vi "Lockin.Low Pass Filter Bank.vi"(6 "Butterworth? [T]":bool=TRUE, 8 "error in (no error)":errorcluster, 10 "WFms in":waveform(dbl)[](array[waveform]), 11 "DSP in":refnum<class "DSP.lvclass">) -> (0 "error out":errorcluster, 2 "Wfms out":waveform(dbl)[](array[waveform]))   [LabVIEW 2019, in "DSP.lvclass"]
uses:
  DSP.lvclass
  DSP.lvclass/DSP.ctl
  Create Low Pass RC Filter (FGV).vi
  Create Low Pass Filter (FGV).vi
  DFD Filter Array.vi
  Waveform.Attributes/Waveform.Attributes.lvlib
panel:
  out "DSP out":refnum<class "DSP.lvclass">
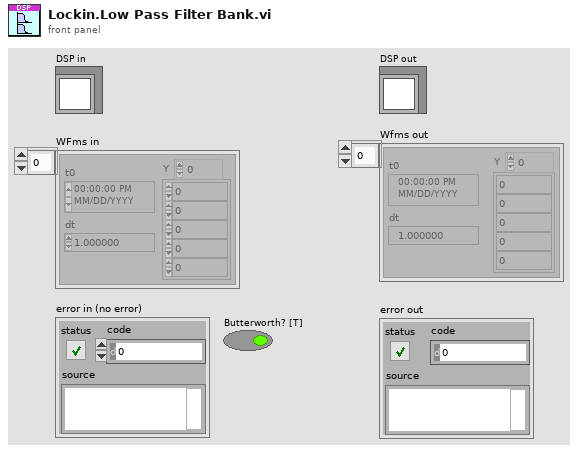
[diagram p1: front panel]
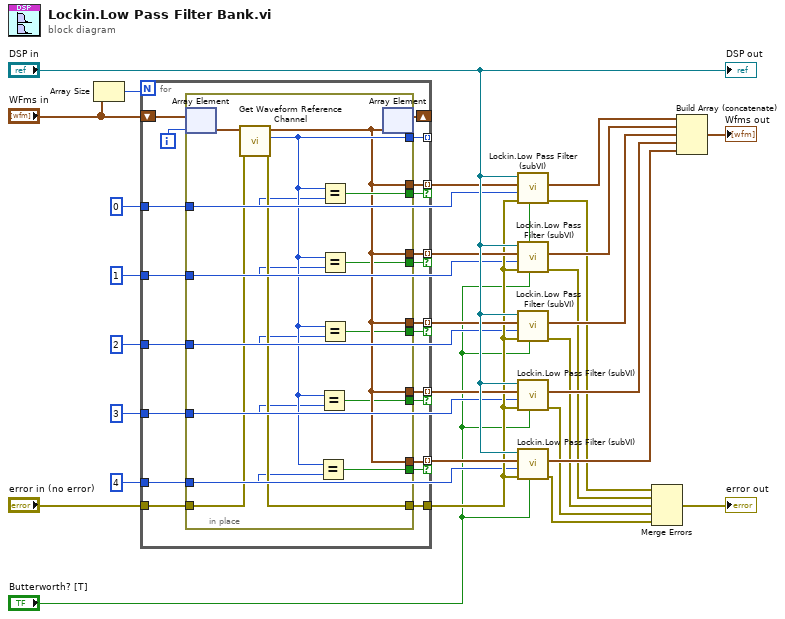
[diagram p0: block diagram]
diagram:
  w6 = 4 ("y")
  w5 = 3 ("y")
  w4 = 2 ("y")
  w3 = 1 ("y")
  w2 = 0 ("y")
  n1 = Array Size(array="WFms in") -> (size(s)=w26:i32)
  n2 = for {
    N: w26 -> [_]
    shift-right: [w44] -> _
    shift-left: "WFms in" -> [w48]
    tunnel: [w45] -> _ mode=indexing
    tunnel: "error in (no error)" -> [w47]
    tunnel: [w46] -> w7
    tunnel: [w43] -> w12 mode=indexing if=w42
    tunnel: [w41] -> w11 mode=indexing if=w34
    tunnel: [w40] -> w10 mode=indexing if=w35
    tunnel: [w39] -> w9 mode=indexing if=w36
    tunnel: [w38] -> w8 mode=indexing if=w37
    tunnel: w6 -> [w33]
    tunnel: w5 -> [w32]
    tunnel: w4 -> [w31]
    tunnel: w3 -> [w30]
    tunnel: w2 -> [w29]
    i -> [w49]
    n3 = in-place {
      in-place-border: w47 -> [w63]
      in-place-border: [w62] -> w46
      in-place-border: [w61] -> w45
      in-place-border: [w59] -> w43
      in-place-border: [w60] -> w42
      in-place-border: [w59] -> w41
      in-place-border: [w59] -> w40
      in-place-border: [w59] -> w39
      in-place-border: [w59] -> w38
      in-place-border: [w58] -> w37
      in-place-border: [w57] -> w36
      in-place-border: [w56] -> w35
      in-place-border: [w55] -> w34
      in-place-border: w33 -> [w54]
      in-place-border: w32 -> [w53]
      in-place-border: w31 -> [w52]
      in-place-border: w30 -> [w51]
      in-place-border: w29 -> [w50]
      n4 = in-place-array #1(w48, w49) -> (w64:waveform(dbl))
      n5 = call "Get Waveform Reference Channel.vi"("error in (no error)"=w63, "Reference in"=w64) -> ("error out"=w62:errorcluster, "Reference Channel"=w61:i32, "Reference out"=w59:waveform(dbl))  [unwired: 7 in]
      n6 = Equal?(x=w61, y=w54) -> (x = y?=w58:bool)
      n7 = Equal?(x=w61, y=w53) -> (x = y?=w57:bool)
      n8 = Equal?(x=w61, y=w50) -> (x = y?=w60:bool)
      n9 = Equal?(x=w61, y=w51) -> (x = y?=w55:bool)
      n10 = Equal?(x=w61, y=w52) -> (x = y?=w56:bool)
      n11 = in-place-array #1(w59) -> (w44:waveform(dbl)[])  [unwired: 1 out]
    }
  }
  n12 = call "Lockin.Low Pass Filter (subVI).vi"("Butterworth? [T]"="Butterworth? [T]", "error in (no error)"=w7, "Element Data"=w2, "signal in"=w12, "DSP in"="DSP in") -> ("error out"=w14:errorcluster, "signal out"=w13:waveform(dbl)[])  [unwired: 3 in, 2 out]
  n13 = call "Lockin.Low Pass Filter (subVI).vi"("Butterworth? [T]"="Butterworth? [T]", "error in (no error)"=w7, "Element Data"=w3, "signal in"=w11, "DSP in"="DSP in") -> ("error out"=w18:errorcluster, "signal out"=w19:waveform(dbl)[])  [unwired: 3 in, 2 out]
  n14 = call "Lockin.Low Pass Filter (subVI).vi"("Butterworth? [T]"="Butterworth? [T]", "error in (no error)"=w7, "Element Data"=w4, "signal in"=w10, "DSP in"="DSP in") -> ("error out"=w17:errorcluster, "signal out"=w20:waveform(dbl)[])  [unwired: 3 in, 2 out]
  n15 = call "Lockin.Low Pass Filter (subVI).vi"("Butterworth? [T]"="Butterworth? [T]", "error in (no error)"=w7, "Element Data"=w5, "signal in"=w9, "DSP in"="DSP in") -> ("error out"=w16:errorcluster, "signal out"=w21:waveform(dbl)[])  [unwired: 3 in, 2 out]
  n16 = call "Lockin.Low Pass Filter (subVI).vi"("Butterworth? [T]"="Butterworth? [T]", "error in (no error)"=w7, "Element Data"=w6, "signal in"=w8, "DSP in"="DSP in") -> ("error out"=w15:errorcluster, "signal out"=w22:waveform(dbl)[])  [unwired: 3 in, 2 out]
  n17 = Merge Errors(w14, w18, w17, w16, w15) -> (→"error out":errorcluster)
  n18 = Build Array (concatenate)(w13, w19, w20, w21, w22) -> (→"Wfms out":waveform(dbl)[])
  "DSP out" <- "DSP in"
